vi "broken-wire.vi"() -> ()   [LabVIEW 2024]
panel:
  out "String":string
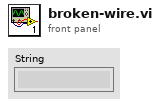
[diagram p1: front panel]
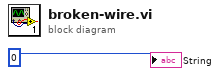
[diagram p0: block diagram]
diagram:
  "String" <- 0
